vi "CSE ISP - vc operations.vi"(6 "cmd":enum16{"before exec", "after exec", "init"}(ring), 8 "error in":errorcluster, 9 "params":T1) -> (0 "error out":errorcluster, 3 "VC Handle":T2=-1)   [LabVIEW 2021]
doc: "::: CalcExpress Toolkit :::\nCopyright (c) 2000-2026 Konstantin Shifershteyn. All rights reserved."
uses:
  vi.lib/addons/CalcExpress/cetypes.llb/VarMan Variable Context Handle.ctl
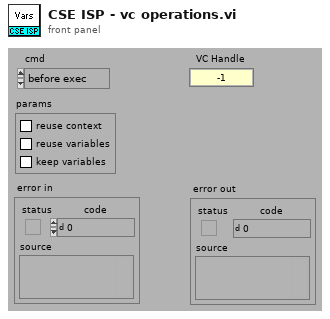
[diagram p1: front panel]
types:
  T1 = cluster{"reuse context":bool, "reuse variables":bool, "keep variables":bool}
  T2 = typedef "VarMan Variable Context Handle.ctl" = i32
  T3 = enum32{"nothing", "reset", "assign name", "get name", "get handle"}
  T4 = typedef "VarMan Variable Info Cluster.ctl" = cluster{"name":string, "alias":string, "type":u32, "history":bool}
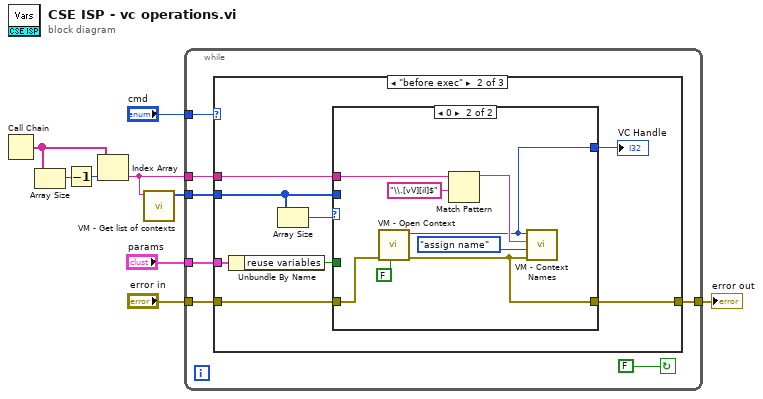
[diagram p0: block diagram]
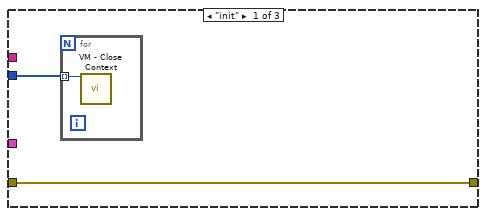
[diagram p2: hidden frame]
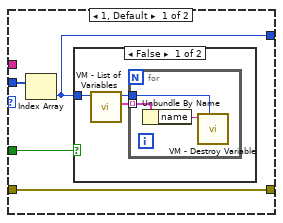
[diagram p3: hidden frame]
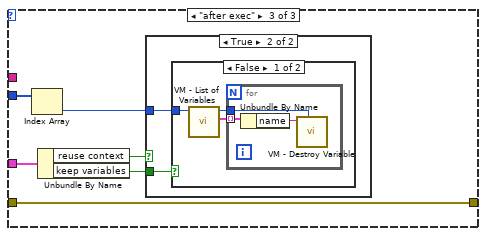
[diagram p5: hidden frame]
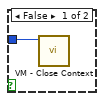
[diagram p6: hidden frame]
diagram:
  n1 = Call Chain() -> (call chain=w5:string[])
  n2 = Array Size(array=w5) -> (size(s)=w4:i32)
  n3 = Decrement(x=w4) -> (x-1=w3:i32)
  n4 = Index Array(array=w5, index=w3) -> (element=w1:string)
  n5 = call "VM - Get list of contexts.vi"("Creator (all contexts)"=w1) -> ("array of VC handles"=w2:T2[])  [unwired: 6 in, 2 out]
  n6 = while {
    tunnel: "cmd" -> [w12]
    tunnel: [w14] -> w7
    tunnel: "error in" -> [w15]
    tunnel: "params" -> [w16]
    tunnel: w1 -> [w11]
    tunnel: w2 -> [w10]
    stop <- FALSE continue-if-true
    n7 = case shown="\"before exec\"" w12 {
      tunnel: w16 -> [_ w24 w51]
      tunnel: w15 -> [w18 w26 w48]
      tunnel: [w18 w27 w48] -> w14
      tunnel: w11 -> [_ w21 _]
      tunnel: w10 -> [w17 w20 w47]
      frame "init" {
        n8 = for {
          tunnel: w17 -> [w19] mode=indexing
          n9 = call "VM - Close Context.vi"("VC Handle"=w19) -> ()  [unwired: 9 in, 2 out]
        }
      }
      frame "before exec" {
        n10 = Unbundle By Name(w24) -> ("reuse variables"=w23:bool)
        n11 = Array Size(array=w20) -> (size(s)=w22:i32)
        n12 = case shown="0" w22 {
          tunnel: w26 -> [w31 w44]
          tunnel: [w31 w43] -> w27
          tunnel: [w28 w40] -> w25
          tunnel: w23 -> [w30 _]
          tunnel: w21 -> [_ w39]
          tunnel: w20 -> [w29 _]
          frame 1, Default {
            n13 = Index Array(array=w29) -> (element=w28:T2)  [unwired: 1 in]
            n14 = case shown="False" w30 {
              tunnel: w28 -> [w32 _]
              frame False {
                n15 = call "VM - List of Variables.vi"("VC Handle"=w32) -> ("variables info"=w33:T4[], "dup VC Handle"=w34:T2)  [unwired: 6 in, 1 out]
                n16 = for {
                  tunnel: w34 -> [w37]
                  tunnel: w33 -> [w35] mode=indexing
                  n17 = Unbundle By Name(w35) -> ("name"=w36:string)
                  n18 = call "VM - Destroy Variable.vi"("VC Handle"=w37, "name_spec"=w36) -> ()  [unwired: 6 in, 4 out]
                }
              }
              frame True {
              }
            }
          }
          frame 0 {
            n19 = call "VM - Open Context.vi"("close loose contexts (F)"=FALSE, "error in"=w44) -> ("error out"=w43:errorcluster, "VC Handle out"=w40:T2)  [unwired: 7 in, 1 out]
            n20 = Match Pattern(string=w39, regular expression="\\.[vV][iI]$") -> (before substring=w41:string)  [unwired: 1 in, 3 out]
            n21 = call "VM - Context Names.vi"("error in"=w43, "action"=T3."assign name", "VC Name"=w41, "VC Handle"=w40) -> ()  [unwired: 2 in, 4 out]
          }
        }
        "VC Handle" <- w25
      }
      frame "after exec" {
        n22 = Index Array(array=w47) -> (element=w46:T2)  [unwired: 1 in]
        n23 = Unbundle By Name(w51) -> ("reuse context"=w50:bool, "keep variables"=w49:bool)
        n24 = case shown="True" w50 {
          tunnel: w46 -> [w52 w53]
          tunnel: w49 -> [_ w54]
          frame False {
            n25 = call "VM - Close Context.vi"("VC Handle"=w52) -> ()  [unwired: 9 in, 2 out]
          }
          frame True {
            n26 = case shown="False" w54 {
              tunnel: w53 -> [w55 _]
              frame False {
                n27 = call "VM - List of Variables.vi"("VC Handle"=w55) -> ("variables info"=w56:T4[], "dup VC Handle"=w57:T2)  [unwired: 6 in, 1 out]
                n28 = for {
                  tunnel: w57 -> [w60]
                  tunnel: w56 -> [w58] mode=indexing
                  n29 = Unbundle By Name(w58) -> ("name"=w59:string)
                  n30 = call "VM - Destroy Variable.vi"("VC Handle"=w60, "name_spec"=w59) -> ()  [unwired: 6 in, 4 out]
                }
              }
              frame True {
              }
            }
          }
        }
      }
    }
  }
  "error out" <- w7
